vi "VIH Project - Control Rule - Filter Out Unused Rules.vi"(11 "Control Rules":T1[](array[typedef])) -> (3 "Control Rules out":T1[](array[typedef]))   [LabVIEW 2014]
doc: "::: VI Helpeks :::\nCopyright (c) 2000-2026 Konstantin Shifershteyn. All rights reserved."
uses:
  _VIH HelpGen.llb/VIH HelpGen Typedef - Cluster - Control Rule.ctl
  _VIH HelpGen.llb/VIH HelpGen Typedef - Enum - Description Mode.ctl
  _VIH HelpGen.llb/VIH HelpGen Typedef - Enum - Default,Enable,Disable.ctl
  _VIH HelpGen.llb/VIH HelpGen Typedef - Cluster - Enum Value Info.ctl
panel:
  # "VI Helpeks\nCopyright (c) 2012-2026 Konstantin Shifershteyn"
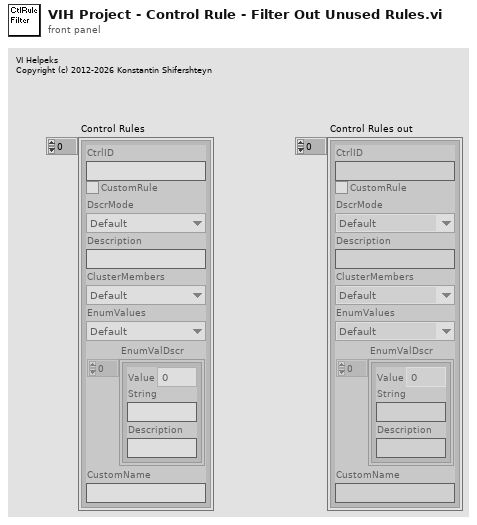
[diagram p1: front panel]
types:
  T1 = typedef "VIH HelpGen Typedef - Cluster - Control Rule.ctl" = cluster{"CtrlID":string, "CustomRule":bool, "DscrMode":T2, "Description":string, "ClusterMembers":T3, "EnumValues":T3, "EnumValDscr":T4[], "CustomName":string}
  T2 = typedef "VIH HelpGen Typedef - Enum - Description Mode.ctl" = enum16{"Default", "Description", "Description1", "Description2", "Custom", "None"}
  T3 = typedef "VIH HelpGen Typedef - Enum - Default,Enable,Disable.ctl" = enum16{"Default", "Enable", "Disable"}
  T4 = typedef "VIH HelpGen Typedef - Cluster - Enum Value Info.ctl" = cluster{"Value":ext, "String":string, "Description":string}
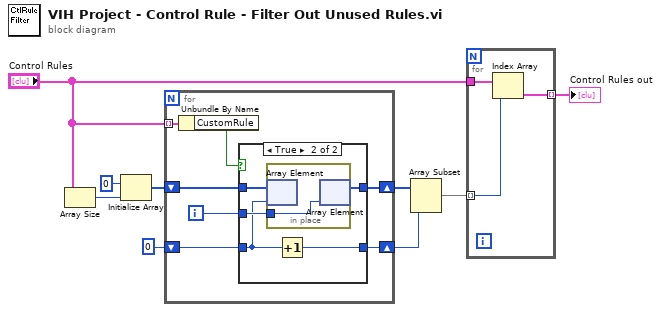
[diagram p0: block diagram]
diagram:
  n1 = Array Size(array="Control Rules") -> (size(s)=w9:i32)
  n2 = Initialize Array(0, w9) -> (w7:i32[])
  n3 = for {
    tunnel: "Control Rules" -> [w16] mode=indexing
    shift-right: [w13] -> w5
    shift-left: w7 -> [w15]
    shift-right: [w11] -> w4
    shift-left: 0 -> [w12]
    i -> [w14]
    n4 = Unbundle By Name(w16) -> ("CustomRule"=w10:bool)
    n5 = case shown="True" w10 {
      tunnel: w15 -> [w18 w23]
      tunnel: w14 -> [_ w22]
      tunnel: [w18 w21] -> w13
      tunnel: w12 -> [w17 w20]
      tunnel: [w17 w19] -> w11
      frame False {
      }
      frame True {
        n6 = in-place {
          in-place-border: w22 -> [w24]
          n7 = in-place-array #1(w23, w20) -> ()  [unwired: 1 out]
          n8 = in-place-array #1(w24) -> (w21:i32[])  [unwired: 1 out]
        }
        n9 = Increment(x=w20) -> (x+1=w19:i32)
      }
    }
  }
  n10 = Array Subset(array=w5, length=w4) -> (w3:i32[])  [unwired: 1 in]
  n11 = for {
    tunnel: "Control Rules" -> [w27]
    tunnel: w3 -> [w26] mode=indexing
    tunnel: [w25] -> w1 mode=indexing
    n12 = Index Array(array=w27, index=w26) -> (element=w25:T1)
  }
  "Control Rules out" <- w1
